vi "copy HO Prameters.vi"(8 "error in (no error)":errorcluster caption="에러 입력(에러 없음)", 11 "NR 입력":refnum<class "NR.lvclass">) -> (0 "error out":errorcluster caption="에러 출력", 3 "NR 출력":refnum<class "NR.lvclass">)   [LabVIEW 2023, in "ANRITSU Call Box.lvlib" / "NR.lvclass"]
uses:
  NR.lvclass
  NR.lvclass/NR.ctl
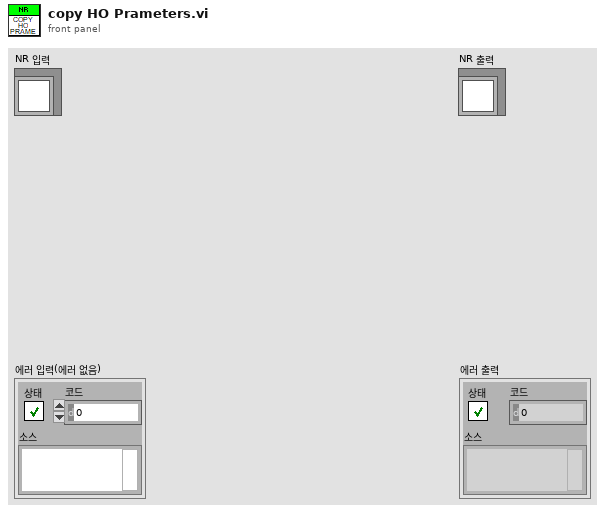
[diagram p1: front panel]
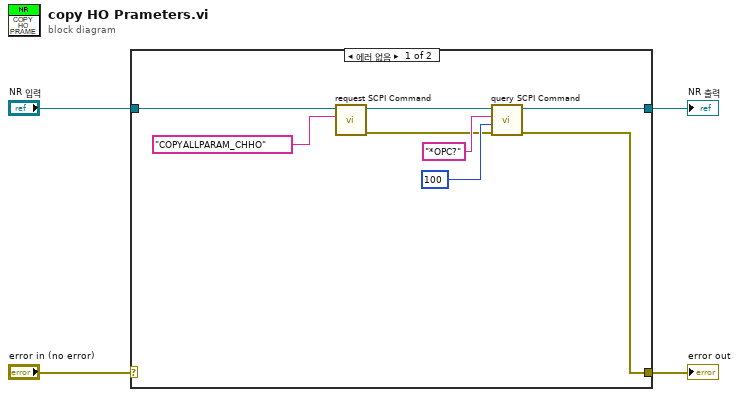
[diagram p0: block diagram]
diagram:
  n1 = case shown="에러 없음" "error in (no error)" {
    selector: "error in (no error)" -> [_ w14]
    tunnel: [w5 w14] -> w3
    tunnel: [w7 w13] -> w1
    tunnel: "NR 입력" -> [w12 w13]
    frame No Error {
      n2 = call "request SCPI Command.vi"("SCPI Command"="COPYALLPARAM_CHHO", "NR in"=w12) -> ("error out"=w6:errorcluster, "NR out"=w10:refnum<class "NR.lvclass">)  [unwired: 8 in]
      n3 = call "query SCPI Command.vi"("error in (no error)"=w6, "Read Buffer Length"=u32 100, "SCPI Command"="*OPC?", "NR in"=w10) -> ("error out"=w5:errorcluster, "NR out"=w7:refnum<class "NR.lvclass">)  [unwired: 5 in, 1 out]
    }
    frame Error {
    }
  }
  "error out" <- w3
  "NR 출력" <- w1
